vi "compera user.vi"(8 "error in (no error)":errorcluster, 10 "输入 1":string="Debug", 11 "connection reference":T1) -> (0 "error out":errorcluster, 2 "data":string[][](array[string]), 3 "connection reference 2":T1)   [LabVIEW 2018, in "login.lvlib"]
uses:
  login.lvlib
  <vilib>/addons/database/Connection.llb/Conn ObjectReference.ctl
  <vilib>/addons/database/Connection.llb/Conn Execute.vi
  <vilib>/addons/database/Recordset.llb/Rec Fetch Recordset Data (R).vi
  <vilib>/addons/database/Recordset.llb/Rec Destroy - Connection.vi
  <vilib>/addons/database/_DB Variant To Data/Database Variant To Data.xnode
  <vilib>/addons/database/NI_Database_API.lvlib
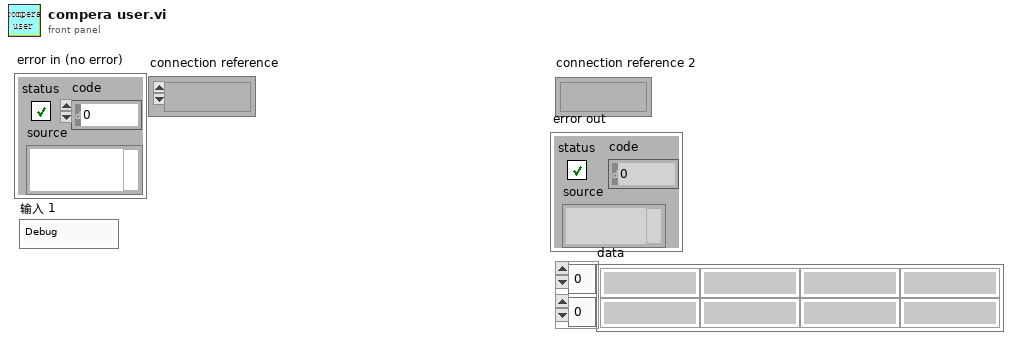
[diagram p1: front panel]
types:
  T1 = typedef "NI_Database_API.lvlib/Conn ObjectReference.ctl" = refnum<k1>
  T2 = typedef "NI_Database_API.lvlib/Rec ObjectReference.ctl" = refnum<k1>
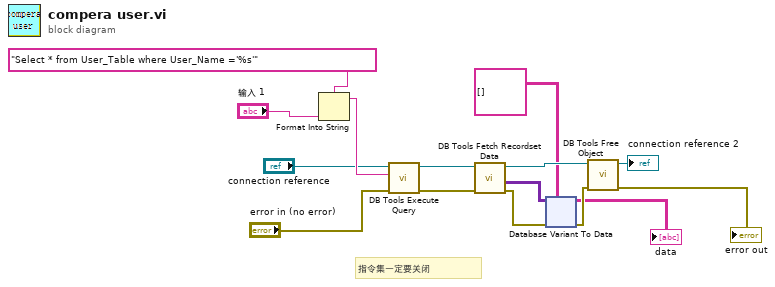
[diagram p0: block diagram]
diagram:
  # "指令集一定要关闭"
  n1 = Format Into String(format string="Select * from User_Table where User_Name ='%s'" ("SQL query"), "输入 1") -> (resulting string=w2:string)  [unwired: 2 in, 1 out]
  n2 = call-poly <vilib>:"DB Tools Execute Query.vi"("error in (no error)"="error in (no error)", "SQL query"=w2, "connection reference"="connection reference") -> ("error out"=w15:errorcluster, "recordset reference"=w13:T2)  [unwired: 5 in]
  n3 = call-poly <vilib>:"DB Tools Fetch Recordset Data.vi"("error in (no error)"=w15, "recordset reference"=w13) -> ("error out"=w9:errorcluster, "recordset data"=w14:variant[][], "recordset reference out"=w7:T2)  [unwired: 3 in]
  n4 = xnode "Database Variant To Data"("database variant"=w14, "error in (no error)"=w9, "type"=string[][] []) -> ("data"=→"data":string[][], "error out"=w8:errorcluster)
  n5 = call-poly <vilib>:"DB Tools Free Object.vi"("error in (no error)"=w8, "recordset reference"=w7) -> ("error out"=→"error out":errorcluster, "connection reference"=→"connection reference 2":T1)  [unwired: 8 in]
